vi "tdms selection.vi"(6 "error in":errorcluster, 8 "string":string="tdms", 11 "Filename List":string[](array[string])) -> (0 "size(s)":i32, 3 "Array 2":string[](array[string]), 4 "error out":errorcluster)   [LabVIEW 2018]
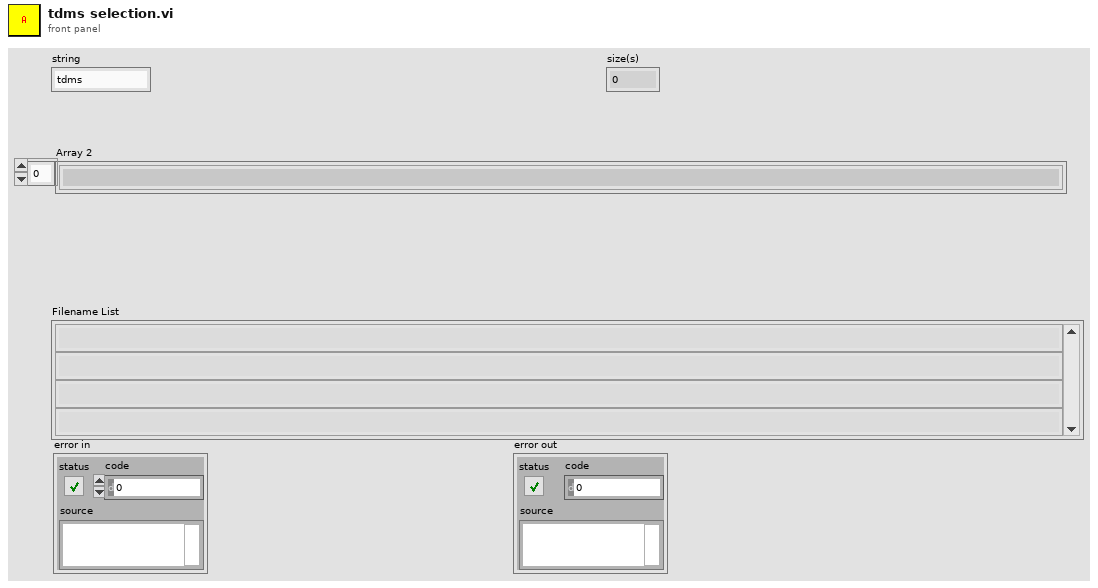
[diagram p1: front panel]
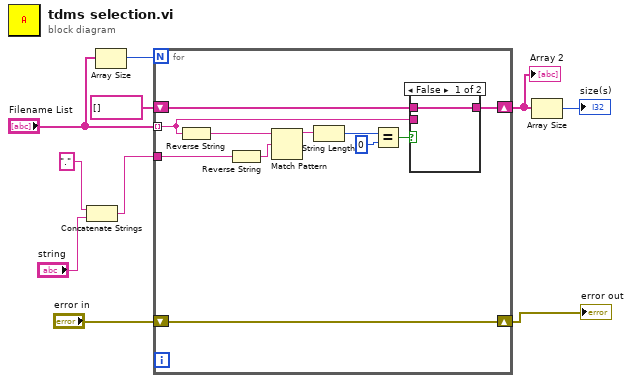
[diagram p0: block diagram]
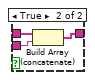
[diagram p2: hidden frame]
diagram:
  n1 = Concatenate Strings("." ("string"), "string") -> (w5:string)
  n2 = Array Size(array="Filename List") -> (size(s)=w10:i32)
  n3 = for {
    N: w10 -> [_]
    tunnel: "Filename List" -> [w15] mode=indexing
    shift-right: [w14] -> w7
    shift-left: string[] [] -> [w13]
    tunnel: w5 -> [w12]
    shift-right: [w11] -> w1
    shift-left: "error in" -> [w11]
    n4 = Reverse String(1:w15) -> (0:w21:string)
    n5 = Reverse String(1:w12) -> (0:w20:string)
    n6 = Match Pattern(string=w21, regular expression=w20) -> (before substring=w19:string)  [unwired: 1 in, 3 out]
    n7 = String Length(string=w19) -> (length=w18:i32)
    n8 = Equal?(x=w18, y=0) -> (x = y?=w16:bool)
    n9 = case shown="False" w16 {
      tunnel: w15 -> [_ w25]
      tunnel: [w22 w24] -> w14
      tunnel: w13 -> [w22 w23]
      frame False {
      }
      frame True {
        n10 = Build Array (concatenate)(w23, w25) -> (w24:string[])
      }
    }
  }
  "Array 2" <- w7
  "error out" <- w1
  n11 = Array Size(array=w7) -> (size(s)=→"size(s)":i32)
